vi "NR Call Process.vi"(8 "error in (no error)":errorcluster caption="에러 입력(에러 없음)", 10 "NR Call Process Param":T1, 11 "Instrument Manager 입력":refnum<class "Instrument Manager.lvclass">) -> (0 "error out":errorcluster caption="에러 출력", 3 "Instrument Manager 출력":refnum<class "Instrument Manager.lvclass">)   [LabVIEW 2023, in "Instrument Manager.lvclass"]
uses:
  Instrument Manager.lvclass
  Type Definition/NR Call Process Param.ctl
  Module/ANRITSU Call Box/Type Definition/NR Modulation Type.ctl
  Instrument Manager.lvclass/Instrument Manager.ctl
  Module/ANRITSU Call Box/ANRITSU Call Box.lvlib
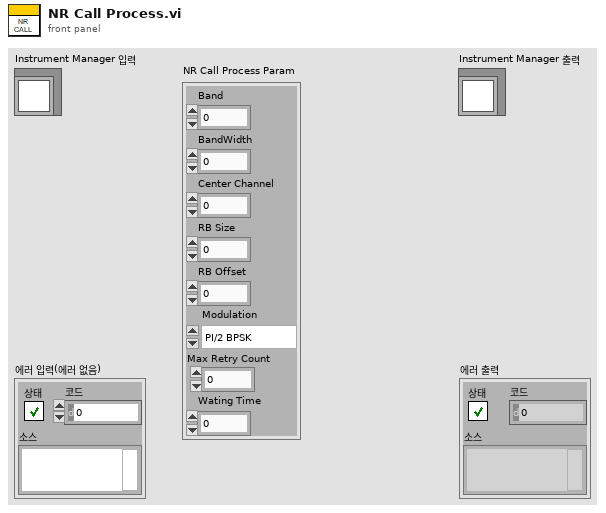
[diagram p1: front panel]
types:
  T1 = typedef "NR Call Process Param.ctl" = cluster{"Band":u32, "BandWidth":u32, "Center Channel":u32, "RB Size":i32, "RB Offset":i32, "Modulation":T2, "Max Retry Count":i32, "Wating Time":i32}
  T2 = typedef "ANRITSU Call Box.lvlib/NR Modulation Type.ctl" = enum16{"PI/2 BPSK", "QPSK", "16QAM", "64QAM", "256QAM"}
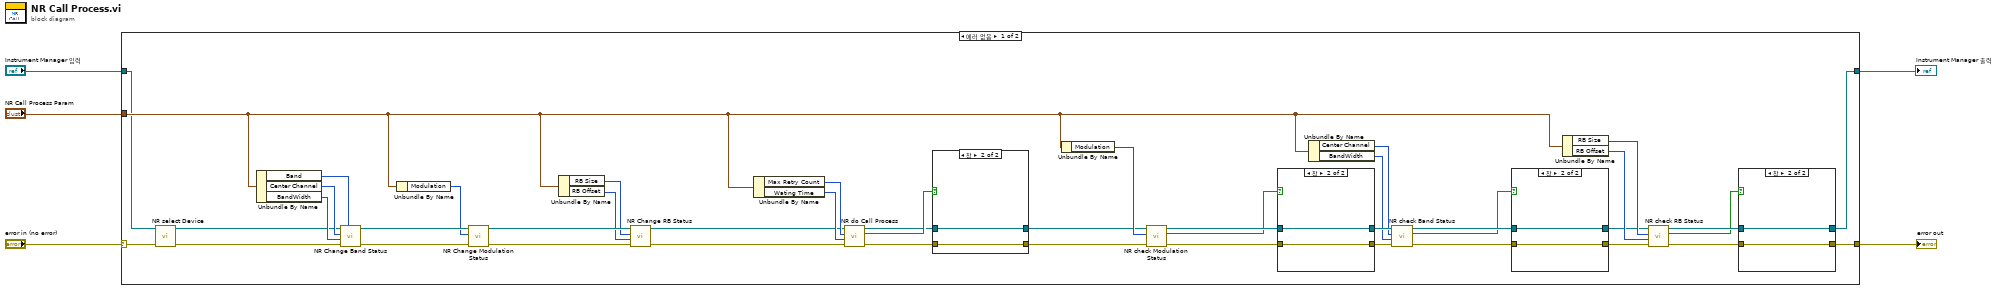
[diagram p0: block diagram]
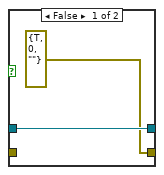
[diagram p2: hidden frame]
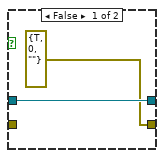
[diagram p3: hidden frame]
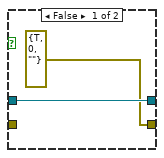
[diagram p4: hidden frame]
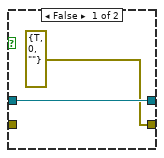
[diagram p5: hidden frame]
diagram:
  n1 = case shown="에러 없음" "error in (no error)" {
    selector: "error in (no error)" -> [w8 w67]
    tunnel: [w37 w67] -> w1
    tunnel: [w36 w66] -> w2
    tunnel: "Instrument Manager 입력" -> [w6 w66]
    tunnel: "NR Call Process Param" -> [w14 _]
    frame No Error {
      n2 = call "NR select Device.vi"("error in (no error)"=w8, "Instrument Manager 입력"=w6) -> ("error out"=w9:errorcluster, "Instrument Manager 출력"=w7:refnum<class "Instrument Manager.lvclass">)  [unwired: 8 in]
      n3 = Unbundle By Name(w14) -> ("Band"=w33:u32, "Center Channel"=w34:u32, "BandWidth"=w35:u32)
      n4 = call "NR Change Band Status.vi"("Operation Band"=w33, "error in (no error)"=w9, "BW (MHz)"=w35, "Center Channel Number"=w34, "Instrument Manager 입력"=w7) -> ("error out"=w48:errorcluster, "Instrument Manager 출력"=w49:refnum<class "Instrument Manager.lvclass">)  [unwired: 5 in]
      n5 = Unbundle By Name(w14) -> ("Modulation"=w32:T2)
      n6 = call "NR Change Modulation Status.vi"("error in (no error)"=w48, "Modulation"=w32, "Instrument Manager 입력"=w49) -> ("error out"=w26:errorcluster, "Instrument Manager 출력"=w25:refnum<class "Instrument Manager.lvclass">)  [unwired: 7 in]
      n7 = Unbundle By Name(w14) -> ("RB Size"=w23:i32, "RB Offset"=w24:i32)
      n8 = call "NR Change RB Status.vi"("error in (no error)"=w26, "RB Offset"=w24, "RB Size"=w23, "Instrument Manager 입력"=w25) -> ("error out"=w13:errorcluster, "Instrument Manager 출력"=w12:refnum<class "Instrument Manager.lvclass">)  [unwired: 6 in]
      n9 = Unbundle By Name(w14) -> ("Max Retry Count"=w15:i32, "Wating Time"=w16:i32)
      n10 = call "NR do Call Process.vi"("error in (no error)"=w13, "Waiting Time"=w16, "Max Retry Count"=w15, "Instrument Manager 입력"=w12) -> ("error out"=w17:errorcluster, "Connected?"=w19:bool, "Instrument Manager 출력"=w18:refnum<class "Instrument Manager.lvclass">)  [unwired: 5 in]
      n11 = case shown="참" w19 {
        tunnel: w18 -> [w51 w53]
        tunnel: [w51 w53] -> w10
        tunnel: [errorcluster {"status"=TRUE, "code"=0, "source"=""} ("error out") w52] -> w11
        tunnel: w17 -> [_ w52]
        frame False {
        }
        frame True {
        }
      }
      n12 = Unbundle By Name(w14) -> ("Modulation"=w31:T2)
      n13 = call "NR check Modulation Status.vi"("error in (no error)"=w11, "Modulation"=w31, "Instrument Manager 입력"=w10) -> ("error out"=w46:errorcluster, "Success?"=w41:bool, "Instrument Manager 출력"=w47:refnum<class "Instrument Manager.lvclass">)  [unwired: 6 in]
      n14 = case shown="참" w41 {
        tunnel: w47 -> [w63 w65]
        tunnel: [w63 w65] -> w45
        tunnel: [errorcluster {"status"=TRUE, "code"=0, "source"=""} ("error out") w64] -> w44
        tunnel: w46 -> [_ w64]
        frame False {
        }
        frame True {
        }
      }
      n15 = Unbundle By Name(w14) -> ("Center Channel"=w29:u32, "BandWidth"=w30:u32)
      n16 = call "NR check Band Status.vi"("error in (no error)"=w44, "BW (MHz)"=w30, "Center Channel Number"=w29, "Instrument Manager 입력"=w45) -> ("error out"=w43:errorcluster, "Success?"=w22:bool, "Instrument Manager 출력"=w42:refnum<class "Instrument Manager.lvclass">)  [unwired: 5 in]
      n17 = case shown="참" w22 {
        tunnel: w42 -> [w59 w61]
        tunnel: [w59 w61] -> w21
        tunnel: [errorcluster {"status"=TRUE, "code"=0, "source"=""} ("error out") w60] -> w20
        tunnel: w43 -> [_ w60]
        frame False {
        }
        frame True {
        }
      }
      n18 = Unbundle By Name(w14) -> ("RB Size"=w27:i32, "RB Offset"=w28:i32)
      n19 = call "NR check RB Status.vi"("error in (no error)"=w20, "RB Offset"=w28, "RB Size"=w27, "Instrument Manager 입력"=w21) -> ("error out"=w39:errorcluster, "Success?"=w38:bool, "Instrument Manager 출력"=w40:refnum<class "Instrument Manager.lvclass">)  [unwired: 5 in]
      n20 = case shown="참" w38 {
        tunnel: w40 -> [w55 w57]
        tunnel: [w55 w57] -> w36
        tunnel: [errorcluster {"status"=TRUE, "code"=0, "source"=""} ("error out") w56] -> w37
        tunnel: w39 -> [_ w56]
        frame False {
        }
        frame True {
        }
      }
    }
    frame Error {
    }
  }
  "error out" <- w1
  "Instrument Manager 출력" <- w2
